vi "Untitled 2.vi"() -> ()   [LabVIEW 2018]
panel:
  out "Waveform Chart":dbl(graph)
  out "String 2":string
  in  "String":string
  out "Boolean 2":bool
  in  "Boolean":bool
  out "output 3":u16
  in  "Input1 2":u16
  out "Output2":i16
  in  "Input1":i32
  out "output":dbl
  in  "Input":dbl
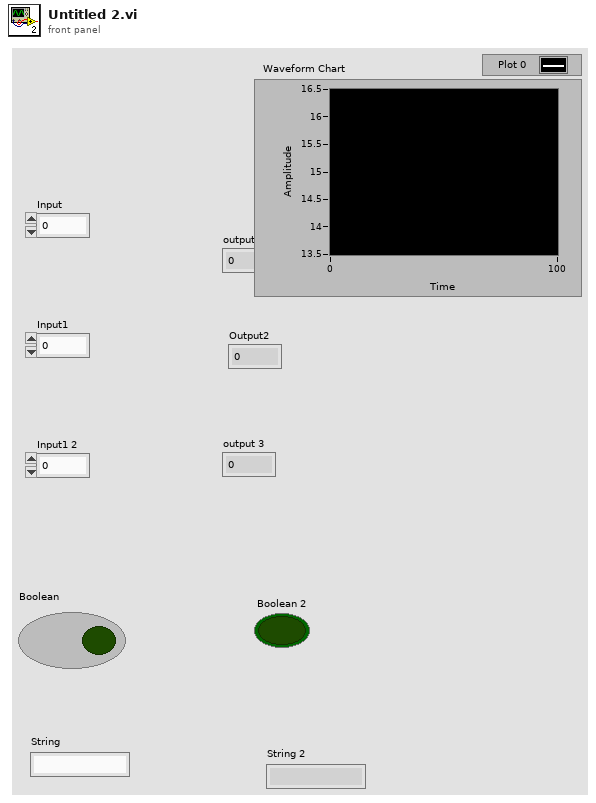
[diagram p1: front panel]
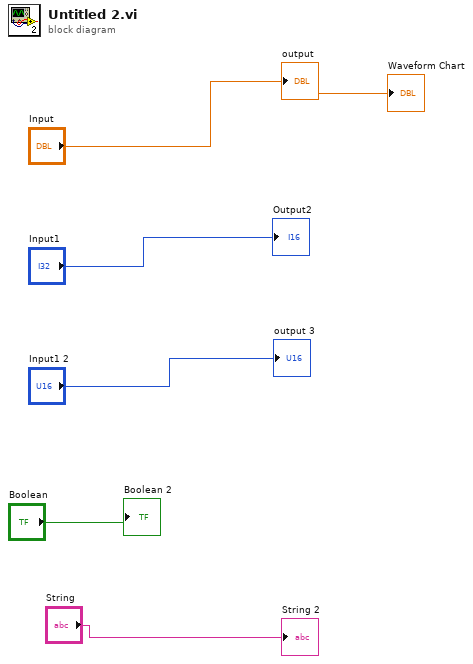
[diagram p0: block diagram]
diagram:
  "output" <- "Input"
  "Output2" <- "Input1"
  "output 3" <- "Input1 2"
  "Boolean 2" <- "Boolean"
  "String 2" <- "String"
  "Waveform Chart" <- "Input"
